vi "Get VI Path for Response Message.vi"(8 "error in (no error)":errorcluster, 11 "Process Path":path) -> (0 "error out":errorcluster, 3 "Path":path)   [LabVIEW 2020, in "Method Generation.lvlib" / "Getter Generator.lvclass"]
uses:
  Getter Generator.lvclass
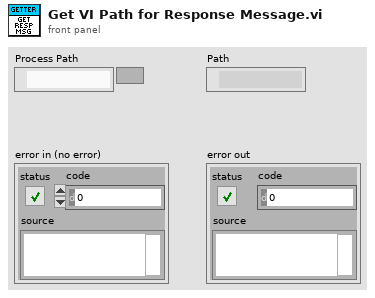
[diagram p1: front panel]
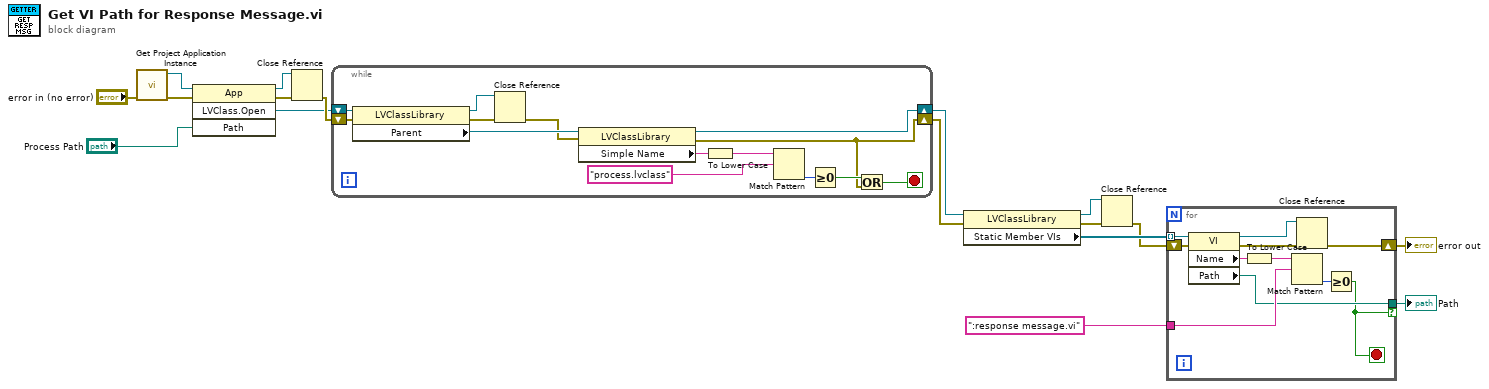
[diagram p0: block diagram]
diagram:
  n1 = call "Get Project Application Instance.vi"("error in (no error)"="error in (no error)") -> ("error out"=w6:errorcluster, "Application out"=w5:refnum<vi>)  [unwired: 9 in]
  n2 = invoke class="App" method="LVClass.Open"(reference=w5, error in=w6, "Path"="Process Path") -> (reference out=w8:refnum<vi>, error out=w7:errorcluster, "LVClass.Open"=w14:refnum<vi>)  [unwired: 1 in, 1 out]
  n3 = Close Reference(reference=w8, error in (no error)=w7) -> (error out=w15:errorcluster)
  n4 = while {
    shift-right: [w29] -> w16
    shift-left: w14 -> [w31]
    shift-right: [w20] -> w3
    shift-left: w15 -> [w27]
    stop <- w21 stop-if-true
    n5 = property class="LVClassLibrary"(reference=w31, error in=w27) -> (reference out=w18:refnum<vi>, error out=w28:errorcluster, "Parent"=w30:refnum<vi>)
    n6 = Close Reference(reference=w18, error in (no error)=w28) -> (error out=w19:errorcluster)
    n7 = property class="LVClassLibrary"(reference=w30, error in=w19) -> (reference out=w29:refnum<vi>, error out=w20:errorcluster, "Simple Name"=w26:string)
    n8 = To Lower Case(string=w26) -> (all lower case string=w25:string)
    n9 = Match Pattern(string=w25, regular expression="process.lvclass") -> (offset past match=w22:i32)  [unwired: 1 in, 3 out]
    n10 = Greater Or Equal To 0?(x=w22) -> (x >= 0?=w23:bool)
    n11 = Or(x=w23, y=w20) -> (x .or. y?=w21:bool)
  }
  n12 = property class="LVClassLibrary"(reference=w16, error in=w3) -> (reference out=w13:refnum<vi>, error out=w12:errorcluster, "Static Member VIs"=w10:refnum<vi>[])
  n13 = Close Reference(reference=w13, error in (no error)=w12) -> (error out=w2:errorcluster)
  n14 = for {
    tunnel: w10 -> [w42] mode=indexing
    tunnel: ":response message.vi" -> [w41]
    tunnel: [w40] -> w17 if=w34
    shift-right: [w32] -> w1
    shift-left: w2 -> [w33]
    stop <- w34 stop-if-true
    n15 = property class="VI"(reference=w42, error in=w33) -> (reference out=w38:refnum<vi>, error out=w39:errorcluster, "Name"=w37:string, "Path"=w40:path)
    n16 = To Lower Case(string=w37) -> (all lower case string=w35:string)
    n17 = Match Pattern(string=w35, regular expression=w41) -> (offset past match=w36:i32)  [unwired: 1 in, 3 out]
    n18 = Close Reference(reference=w38, error in (no error)=w39) -> (error out=w32:errorcluster)
    n19 = Greater Or Equal To 0?(x=w36) -> (x >= 0?=w34:bool)
  }
  "Path" <- w17
  "error out" <- w1
